vi "Send Inband Response.vi"(8 "error in (no error)":errorcluster caption="에러 입력(에러 없음)", 9 "Amplitude":dbl, 10 "id":string, 11 "Instrument Manager 입력":refnum<class "Instrument Manager.lvclass">) -> (0 "error out":errorcluster caption="에러 출력", 3 "Instrument Manager 출력":refnum<class "Instrument Manager.lvclass">)   [LabVIEW 2023, in "Instrument Manager.lvclass"]
uses:
  Instrument Manager.lvclass
  Instrument Manager.lvclass/Instrument Manager.ctl
  Error Response.ctl
  InBand Response.ctl
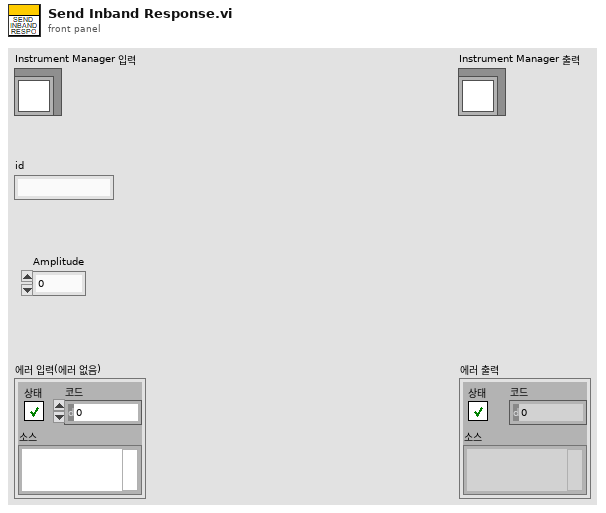
[diagram p1: front panel]
types:
  T1 = typedef "Instrument Manager.lvclass/InBand Response.ctl" = cluster{"type":string, "id":string, "status":string, "Result":cluster{"Amplitude":dbl}}
  T2 = cluster{"Reader Q":refnum<queue>, "Writer Q":refnum<queue>}
  T3 = typedef "Instrument Manager.lvclass/Error Response.ctl" = cluster{"type":string, "id":string, "status":string, "error out":errorcluster}
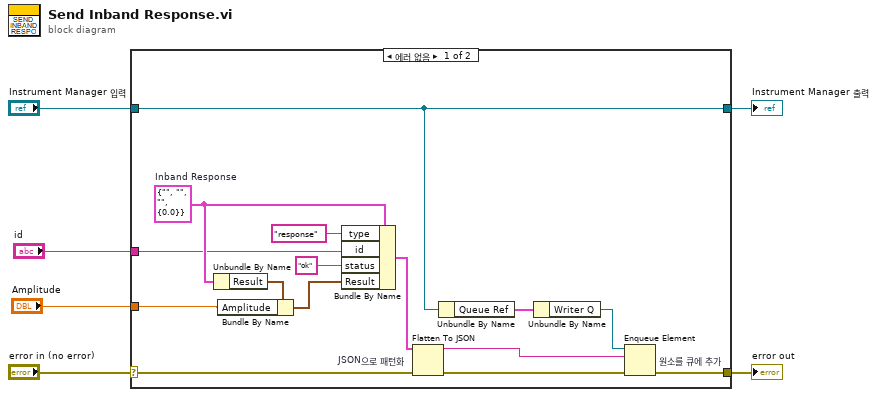
[diagram p0: block diagram]
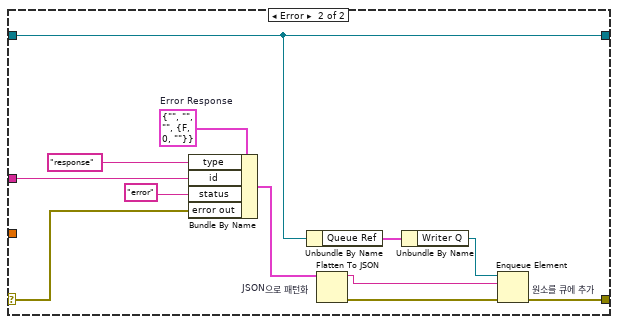
[diagram p2: hidden frame]
diagram:
  n1 = case shown="에러 없음" "error in (no error)" {
    selector: "error in (no error)" -> [w12 w26]
    tunnel: [w10 w27] -> w5
    tunnel: [w9 w24] -> w3
    tunnel: "Instrument Manager 입력" -> [w9 w24]
    tunnel: "id" -> [w17 w25]
    tunnel: "Amplitude" -> [w8 _]
    frame No Error {
      w18 = T1 {"type"="", "id"="", "status"="", "Result"={"Amplitude"=0.0}}  # Inband Response
      n2 = Unbundle By Name(w18) -> ("Result"=w20:cluster{"Amplitude":dbl})
      n3 = Bundle By Name(cluster=w20, "Amplitude"=w8) -> (w19:cluster{"Amplitude":dbl})
      n4 = Bundle By Name(cluster=w18, "type"="response", "id"=w17, "status"="ok", "Result"=w19) -> (w13:T1)
      n5 = Flatten To JSON "JSON으로 패턴화"(anything=w13, error in (no error)=w12) -> (JSON string=w14:string, 11:w11:errorcluster)  [unwired: 1 in]
      n6 = Unbundle By Name(w9) -> ("Queue Ref"=w16:T2)
      n7 = Unbundle By Name(w16) -> ("Writer Q"=w15:refnum<queue>)
      n8 = Enqueue Element "원소를 큐에 추가"(queue=w15, element=w14, error in (no error)=w11) -> (error out=w10:errorcluster)  [unwired: 1 in, 2 out]
    }
    frame Error {
      w33 = T3 {"type"="", "id"="", "status"="", "error out"={"status"=FALSE, "code"=0, "source"=""}}  # Error Response
      n9 = Bundle By Name(cluster=w33, "type"="response", "id"=w25, "status"="error", "error out"=w26) -> (w29:T3)
      n10 = Unbundle By Name(w24) -> ("Queue Ref"=w23:T2)
      n11 = Flatten To JSON "JSON으로 패턴화"(anything=w29) -> (JSON string=w32:string, 11:w28:errorcluster)  [unwired: 2 in]
      n12 = Unbundle By Name(w23) -> ("Writer Q"=w22:refnum<queue>)
      n13 = Enqueue Element "원소를 큐에 추가"(queue=w22, element=w32, error in (no error)=w28) -> (error out=w27:errorcluster)  [unwired: 1 in, 2 out]
    }
  }
  "error out" <- w5
  "Instrument Manager 출력" <- w3
